vi "TCP_audio+video.vi"() -> ()   [LabVIEW 2021]
uses:
  <vilib>/sound2/lvsound2.llb/Sampling Mode.ctl
  <vilib>/sound2/lvsound2.llb/Sound Data Format.ctl
  <vilib>/sound2/lvsound2.llb/Sound Output Write (DBL Single).vi
panel:
  out "Video Picture 3":picture
  in  "通道选择":dbl
  out "byte_index":dbl
  out "Waveform Graph 3":waveform(dbl)(graph)
  out "collect_buffer_size 2":i32
  out "image_count":i32
  out "audio_count":i32
  out "bad_head_count":i32
  out "unsigned byte array":u8[](array[numeric])
  out "is_image":bool
  out "payload_u8_size":i32
  out "payload_read_len":u32
  out "is_audio":bool
  out "element 8":u8 format="%x"
  out "element 7":u8 format="%x"
  out "element 6":u8 format="%x"
  out "element 5":u8 format="%x"
  out "element 4":u8 format="%x"
  out "element 3":u8 format="%x"
  out "element 2":u8 format="%x"
  out "element":u8 format="%x"
  out "payload_len":u32
  in  "mode (standard)":T1(ring)
  in  "stop":bool
  in  "端口":dbl=9968.0
  in  "IP地址":string="192.168.2.10"
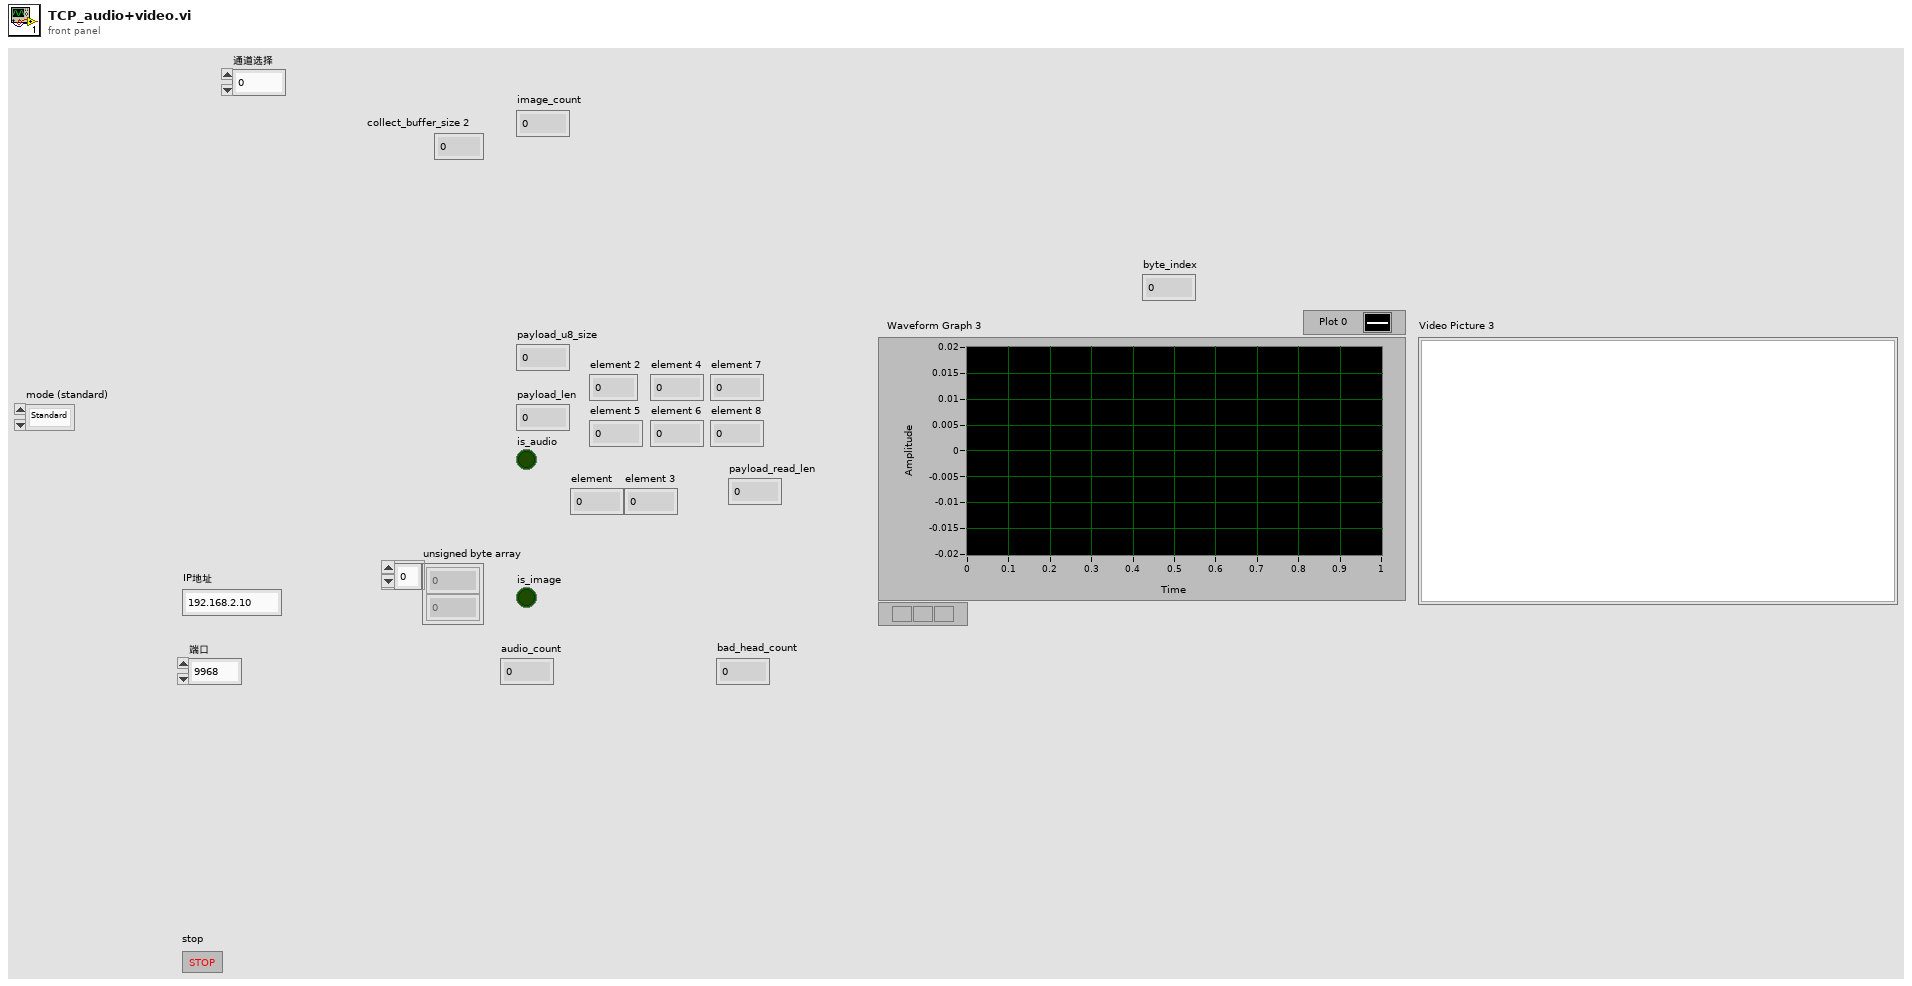
[diagram p1: front panel]
types:
  T1 = enum16{"Standard", "Buffered", "CRLF", "Immediate"}
  T2 = typedef "Sound Data Format.ctl" = cluster{"sample rate (S/s)":dbl, "number of channels":i32, "bits per sample":i32}
  T3 = typedef "Sampling Mode.ctl" = i32
  T4 = typedef "Sound Output Task ID.ctl" = u32
  T5 = enum16{"big-endian, network order", "native, host order", "little-endian"}
  T6 = typedef "imagedata.ctl" = cluster{"image type":i32, "image depth":i32, "image":u8[], "mask":u8[], "colors":u32[], "Rectangle":cluster{"left":i16, "top":i16, "right":i16, "bottom":i16}}
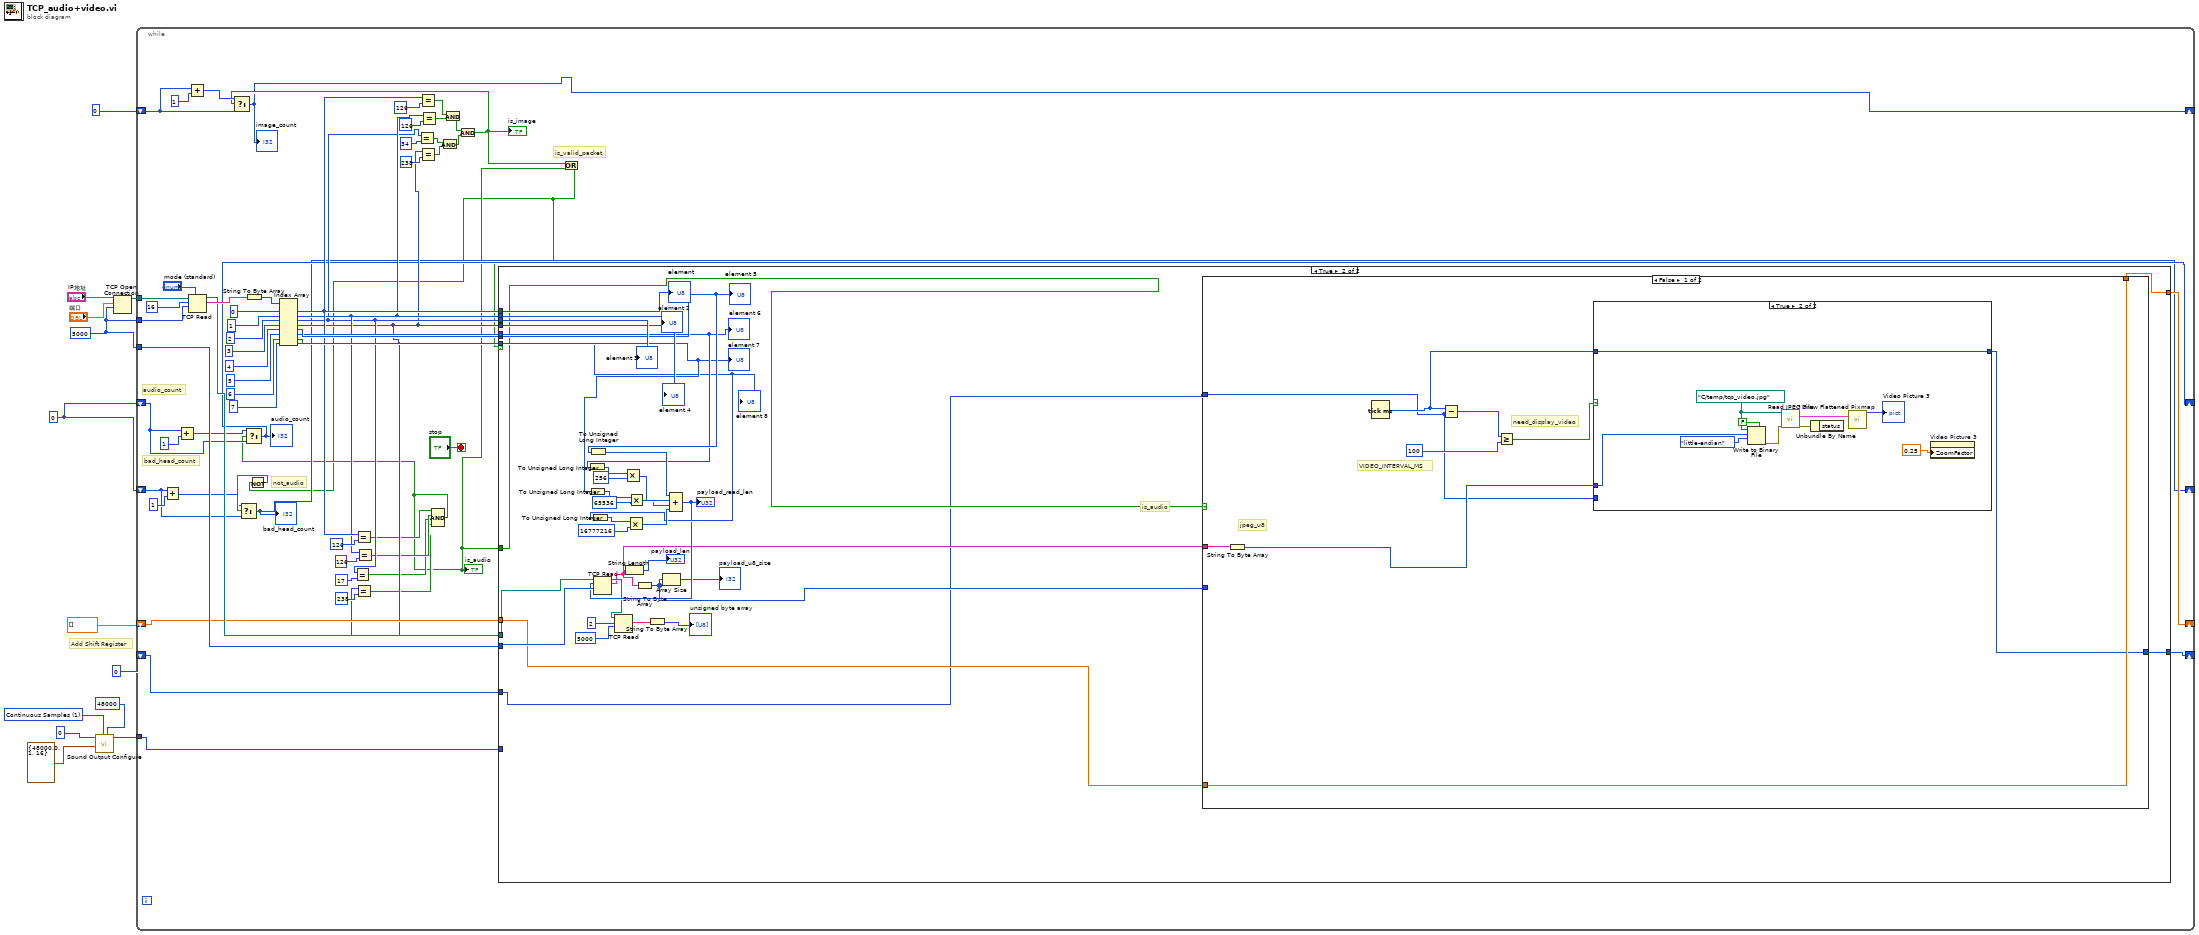
[diagram p0: block diagram]
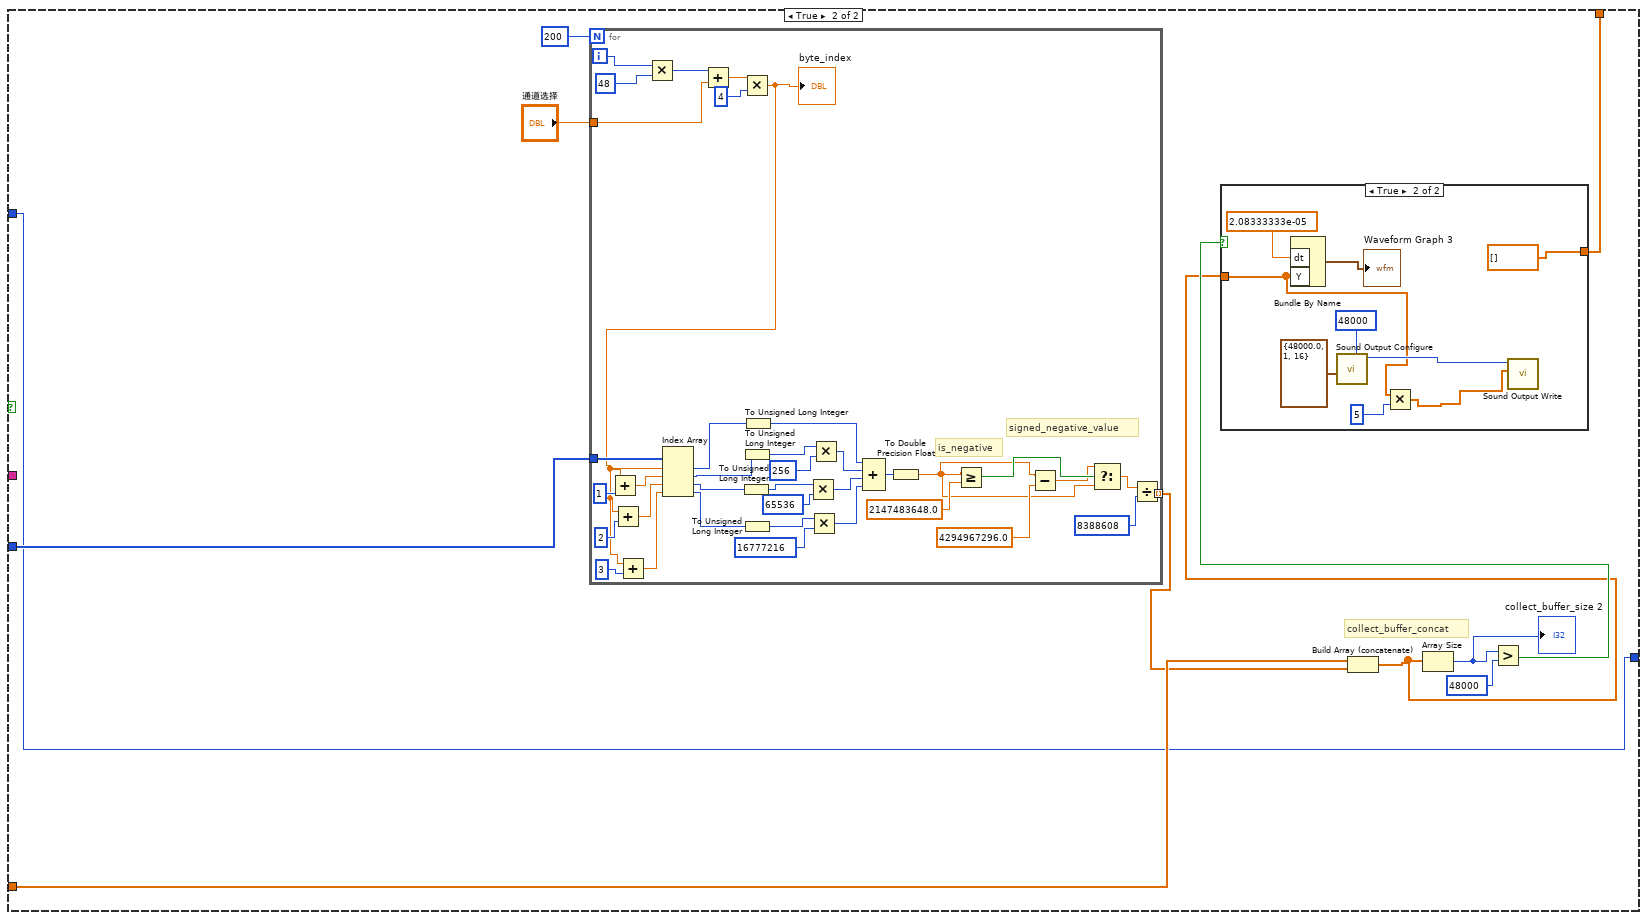
[diagram p4: hidden frame]
diagram:
  w3 = 0
  w7 = T3 1 items=["Finite Samples", "Continuous Samples"] ("sample mode")
  w10 = 5000
  # "Add Shift Register"
  n1 = call <vilib>:"Sound Output Configure.vi"("number of samples/ch"=48000, "sample mode"=w7, "sound format"=T2 {"sample rate (S/s)"=48000.0, "number of channels"=1, "bits per sample"=16}, "device ID"=0) -> ("task ID"=w4:T4)  [unwired: 6 in, 1 out]
  n2 = TCP Open Connection(address="IP地址", remote port or service name="端口", timeout ms (60000)=w10) -> (connection ID=w11:refnum<k5>)  [unwired: 2 in, 1 out]
  n3 = while {
    tunnel: w11 -> [w76]
    tunnel: w10 -> [w74]
    tunnel: w10 -> [w54]
    shift-right: [w50] -> _
    shift-left: dbl[] [] -> [w52]
    tunnel: w4 -> [w51]
    shift-right: [w28] -> _
    shift-left: w3 -> [w29]
    shift-right: [w23] -> _
    shift-left: w3 -> [w24]
    shift-right: [w16] -> _
    shift-left: 0 -> [w20]
    shift-right: [w14] -> _
    shift-left: 0 -> [w15]
    stop <- "stop" stop-if-true
    # "is_valid_packet"
    # "not_audio"
    # "bad_head_count"
    # "audio_count"
    n4 = Add(x=w24, y=1) -> (x+y=w25:i32)
    n5 = Add(x=w29, y=1) -> (x+y=w30:i32)
    n6 = Add(x=w20, y=1) -> (x+y=w21:i32)
    n7 = TCP Read(connection ID=w76, bytes to read=16, 7:"mode (standard)", 9:w74) -> (connection ID out=w53:refnum<k5>, data out=w72:string)  [unwired: 1 in, 1 out]
    n8 = String To Byte Array(string=w72) -> (unsigned byte array=w71:u8[])
    n9 = Index Array(array=w71, index #1=0, index #2=1, index #3=2, index #4=3, index #5=4, index #6=5, index #7=6, index #8=7) -> (element #1=w39:u8, element #2=w38:u8, element #3=w37:u8, element #4=w36:u8, element #5=w62:u8, element #6=w61:u8, element #7=w60:u8, element #8=w59:u8)
    n10 = Equal?(x=w37, y=u8 17) -> (x = y?=w33:bool)
    n11 = Equal?(x=w39, y=u8 126) -> (x = y?=w35:bool)
    n12 = Equal?(x=w36, y=u8 238) -> (x = y?=w32:bool)
    n13 = Equal?(x=w38, y=u8 126) -> (x = y?=w34:bool)
    n14 = Equal?(x=w37, y=u8 34) -> (x = y?=w43:bool)
    n15 = Equal?(x=w39, y=u8 126) -> (x = y?=w45:bool)
    n16 = Equal?(x=w36, y=u8 238) -> (x = y?=w42:bool)
    n17 = Equal?(x=w38, y=u8 126) -> (x = y?=w44:bool)
    n18 = Compound Arithmetic op=AND(w35, w34, w33, w32) -> (w18:bool)
    "is_audio" <- w18
    n19 = Select(t=w30, s=w18, f=w29) -> (s? t:f=w28:i32)
    "audio_count" <- w28
    n20 = And(x=w43, y=w42) -> (x .and. y?=w40:bool)
    n21 = And(x=w45, y=w44) -> (x .and. y?=w41:bool)
    n22 = And(x=w41, y=w40) -> (x .and. y?=w19:bool)
    "is_image" <- w19
    n23 = Select(t=w21, s=w19, f=w20) -> (s? t:f=w16:i32)
    "image_count" <- w16
    n24 = Or(x=w19, y=w18) -> (x .or. y?=w17:bool)
    n25 = Not(x=w17) -> (.not. x?=w26:bool)
    n26 = Select(t=w25, s=w26, f=w24) -> (s? t:f=w23:i32)
    "bad_head_count" <- w23
    n27 = case shown="True" w17 {
      tunnel: w62 -> [_ w97]
      tunnel: w61 -> [_ w96]
      tunnel: w60 -> [_ w95]
      tunnel: w59 -> [_ w94]
      tunnel: w39 -> [_ w114]
      tunnel: w38 -> [_ w113]
      tunnel: w37 -> [_ w112]
      tunnel: w36 -> [_ w111]
      tunnel: w54 -> [_ w110]
      tunnel: w53 -> [_ w109]
      tunnel: w52 -> [w79 w85]
      tunnel: [w79 w84] -> w50
      tunnel: w51 -> [_ _]
      tunnel: w18 -> [_ w86]
      tunnel: w15 -> [w78 w81]
      tunnel: [w78 w80] -> w14
      frame False {
      }
      frame True {
        # "is_audio"
        n28 = To Unsigned Long Integer(number=w96) -> (unsigned 32bit integer=w107:u32)
        n29 = To Unsigned Long Integer(number=w95) -> (unsigned 32bit integer=w105:u32)
        n30 = To Unsigned Long Integer(number=w97) -> (unsigned 32bit integer=w101:u32)
        n31 = To Unsigned Long Integer(number=w94) -> (unsigned 32bit integer=w103:u32)
        n32 = Multiply(x=w107, y=256) -> (x*y=w100:u32)
        n33 = Multiply(x=w103, y=16777216) -> (x*y=w98:u32)
        n34 = Multiply(x=w105, y=65536) -> (x*y=w99:u32)
        n35 = Compound Arithmetic op=ADD(w101, w100, w99, w98) -> (w93:u32)
        "payload_read_len" <- w93
        n36 = TCP Read(connection ID=w109, bytes to read=w93, 9:w110) -> (connection ID out=w91:refnum<k5>, data out=w82:string)  [unwired: 2 in, 1 out]
        n37 = TCP Read(connection ID=w91, bytes to read=2, 9:5000) -> (data out=w88:string)  [unwired: 2 in, 2 out]
        n38 = String Length(string=w82) -> (length=→"payload_len":i32)
        n39 = String To Byte Array(string=w82) -> (unsigned byte array=w83:u8[])
        n40 = String To Byte Array(string=w88) -> (unsigned byte array=→"unsigned byte array":u8[])
        n41 = Array Size(array=w83) -> (size(s)=→"payload_u8_size":i32)
        n42 = case shown="False" w86 {
          tunnel: w85 -> [w123 w141]
          tunnel: [w123 w140] -> w84
          tunnel: w83 -> [_ w137]
          tunnel: w82 -> [w122 _]
          tunnel: w81 -> [w115 w135]
          tunnel: [w116 w135] -> w80
          frame False {
            # "need_display_video"
            # "VIDEO_INTERVAL_MS"
            # "jpeg_u8"
            n43 = String To Byte Array(string=w122) -> (unsigned byte array=w120:u8[])
            n44 = Tick Count (ms)() -> (millisecond timer value=w117:u32)
            n45 = Subtract(x=w117, y=w115) -> (x-y=w121:u32)
            n46 = Greater Or Equal?(x=w121, y=100) -> (x >= y?=w119:bool)
            n47 = case shown="True" w119 {
              tunnel: w120 -> [_ w126]
              tunnel: w117 -> [_ w125]
              tunnel: [w124 w125] -> w116
              tunnel: w115 -> [w124 _]
              frame False {
              }
              frame True {
                w131 = path "C:/temp/tcp_video.jpg" ("file (use dialog)")
                n48 = Write to Binary File(file (use dialog)=w131, data=w126, 5:FALSE ("prepend array or string size? (T)"), 9:T5."little-endian" ("byte order (0:big-endian, network order)")) -> (error out=w134:errorcluster)  [unwired: 2 in, 2 out]
                n49 = call <vilib>:"Read JPEG File.vi"("error in (no error)"=w134, "path to JPEG file"=w131) -> ("error out"=w130:errorcluster, "image data"=w129:T6)  [unwired: 7 in, 1 out]
                n50 = Unbundle By Name(w130) -> ()  [unwired: 1 out]
                n51 = call <vilib>:"Draw Flattened Pixmap.vi"("image data"=w129) -> ("new picture"=→"Video Picture 3":picture)  [unwired: 8 in]
                n52 = property on="Video Picture 3" class="Pict"("ZoomFactor"=0.25) -> ()  [unwired: 2 in, 2 out]
              }
            }
          }
          frame True {
            # "collect_buffer_concat"
            n53 = for {
              N: 200 -> [_]
              tunnel: w137 -> [w176]
              tunnel: "通道选择" -> [w180]
              tunnel: [w148] -> w136 mode=indexing
              i -> [w177]
              # "signed_negative_value"
              # "is_negative"
              n54 = Multiply(x=w177, y=48) -> (x*y=w181:i32)
              n55 = Add(x=w181, y=w180) -> (x+y=w179:dbl)
              n56 = Multiply(x=w179, y=4) -> (x*y=w170:dbl)
              "byte_index" <- w170
              n57 = Add(x=w170, y=1) -> (x+y=w174:dbl)
              n58 = Add(x=w170, y=2) -> (x+y=w172:dbl)
              n59 = Add(x=w170, y=3) -> (x+y=w169:dbl)
              n60 = Index Array(array=w176, index #1=w170, index #2=w174, index #3=w172, index #4=w169) -> (element #1=w168:u8, element #2=w167:u8, element #3=w166:u8, element #4=w165:u8)
              n61 = To Unsigned Long Integer(number=w166) -> (unsigned 32bit integer=w163:u32)
              n62 = To Unsigned Long Integer(number=w167) -> (unsigned 32bit integer=w164:u32)
              n63 = To Unsigned Long Integer(number=w165) -> (unsigned 32bit integer=w162:u32)
              n64 = To Unsigned Long Integer(number=w168) -> (unsigned 32bit integer=w158:u32)
              n65 = Multiply(x=w163, y=65536) -> (x*y=w156:u32)
              n66 = Multiply(x=w162, y=16777216) -> (x*y=w155:u32)
              n67 = Multiply(x=w164, y=256) -> (x*y=w157:u32)
              n68 = Compound Arithmetic op=ADD(w158, w157, w156, w155) -> (w154:u32)
              n69 = To Double Precision Float(number=w154) -> (double precision float=w146:dbl)
              n70 = Greater Or Equal?(x=w146, y=2147483648.0) -> (x >= y?=w152:bool)
              n71 = Subtract(x=w146, y=4294967296.0) -> (x-y=w151:dbl)
              n72 = Select(t=w151, s=w152, f=w146) -> (s? t:f=w150:dbl)
              n73 = Divide(x=w150, y=8388608) -> (x/y=w148:dbl)
            }
            n74 = Build Array (concatenate)(w141, w136) -> (w142:dbl[])
            n75 = Array Size(array=w142) -> (size(s)=w145:i32)
            "collect_buffer_size 2" <- w145
            n76 = Greater?(x=w145, y=48000) -> (0:w143:bool)
            n77 = case shown="True" w143 {
              tunnel: w142 -> [w183 w186]
              tunnel: [w183 dbl[] []] -> w140
              frame False {
              }
              frame True {
                n78 = Bundle By Name("dt"=2.08333333e-05, "Y"=w186) -> (→"Waveform Graph 3":waveform(dbl))  [unwired: 1 in]
                n79 = call <vilib>:"Sound Output Configure.vi"("number of samples/ch"=48000, "sound format"=T2 {"sample rate (S/s)"=48000.0, "number of channels"=1, "bits per sample"=16}) -> ("task ID"=w189:T4)  [unwired: 8 in, 1 out]
                n80 = Multiply(x=w186, y=5 ("bits per sample")) -> (x*y=w184:dbl[])
                n81 = call-poly <vilib>:"Sound Output Write.vi"("data"=w184, "task ID"=w189) -> ()  [unwired: 8 in, 2 out]
              }
            }
          }
        }
        "element" <- w114
        "element 2" <- w113
        "element 3" <- w112
        "element 4" <- w111
        "element 5" <- w97
        "element 6" <- w96
        "element 7" <- w95
        "element 8" <- w94
      }
    }
  }
